vi "binary_string.vi"() -> ()   [LabVIEW 2021]
panel:
  out "string":string
  out "string length":i32
  out "data":u8[](array[numeric])
  out "path":path
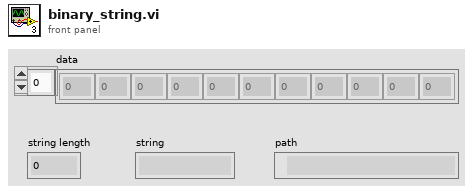
[diagram p1: front panel]
types:
  T1 = enum16{"open", "replace", "create", "open or create", "replace or create", "replace or create with confirmation"}
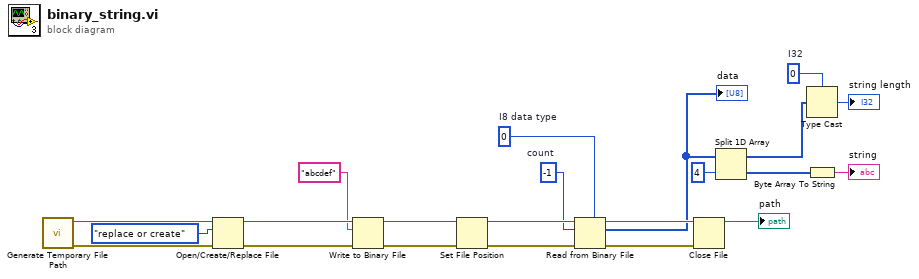
[diagram p0: block diagram]
diagram:
  w5 = 0  # I32
  w8 = -1  # count
  w9 = u8 0  # I8 data type
  n1 = call <vilib>:"Generate Temporary File Path.vi"() -> ("error out"=w15:errorcluster, "Unique Temporary File Path"=w16:path)  [unwired: 10 in]
  n2 = Open/Create/Replace File(file path (use dialog)=w16, error in=w15, operation (0:open)=T1."replace or create") -> (refnum out=w13:refnum<file>, error out=w14:errorcluster)  [unwired: 3 in, 1 out]
  n3 = Write to Binary File(file (use dialog)=w13, data="abcdef", error in=w14) -> (refnum out=w20:refnum<file>, error out=w18:errorcluster)  [unwired: 3 in, 1 out]
  n4 = Set File Position(refnum=w20, error in=w18) -> (refnum out=w19:refnum<file>, error out=w17:errorcluster)  [unwired: 2 in]
  n5 = Read from Binary File(5:w9, 8:w17, 10:w8, 11:w19) -> (0:w21:errorcluster, 2:w7:u8[], 3:w22:refnum<file>)  [unwired: 2 in, 1 out]
  "data" <- w7
  n6 = Close File(refnum=w22, error in=w21) -> (path=→"path":path)  [unwired: 1 out]
  n7 = Split 1D Array(array=w7, index=4) -> (first subarray=w4:u8[], second subarray=w2:u8[])
  n8 = Type Cast(type=w5, x=w4) -> (*(type *) &x=→"string length":i32)
  n9 = Byte Array To String(unsigned byte array=w2) -> (string=→"string":string)
